vi "Sequence.BuildWaveformStep.vi"(7 "FirstIteration":bool, 9 "Current Waveform":waveform(dbl)[](array[waveform]), 10 "Steps":string[](array[string]), 11 "DataPoints":u64) -> (0 "Step Type":T1[](array[typedef]), 1 "IO Points":cluster{"Ramp Pattern":dbl[]}[](array[cluster]), 2 "iStep":bool, 3 "iStep Size":i32)   [LabVIEW 2015, in "Simple Sequence Tools - Shared.lvlib"]
uses:
  Simple Sequence Tools - Shared.lvlib
  Types/Step.Types.ctl
  <vilib>/Analysis/1siggen.llb/Ramp Pattern by Samples.vi
  <vilib>/Analysis/NI_AALBase.lvlib
  <vilib>/measure/NI_MABase.lvlib
panel:
  in  "DataPoints out":u64
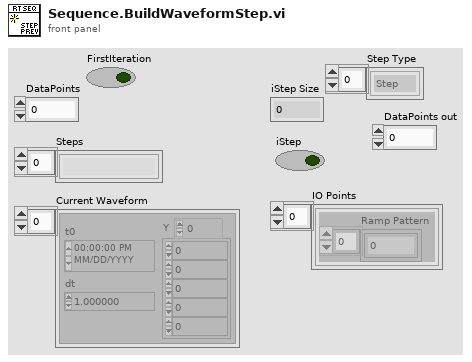
[diagram p1: front panel]
types:
  T1 = typedef "Simple Sequence Tools - Shared.lvlib/Step.Types.ctl" = enum8{"Step", "iStep", "Ramp", "Unchanged", "Unknown", "Sine", "LogSine", "LinearSine", "ForcedRamp", "SquareWave"}
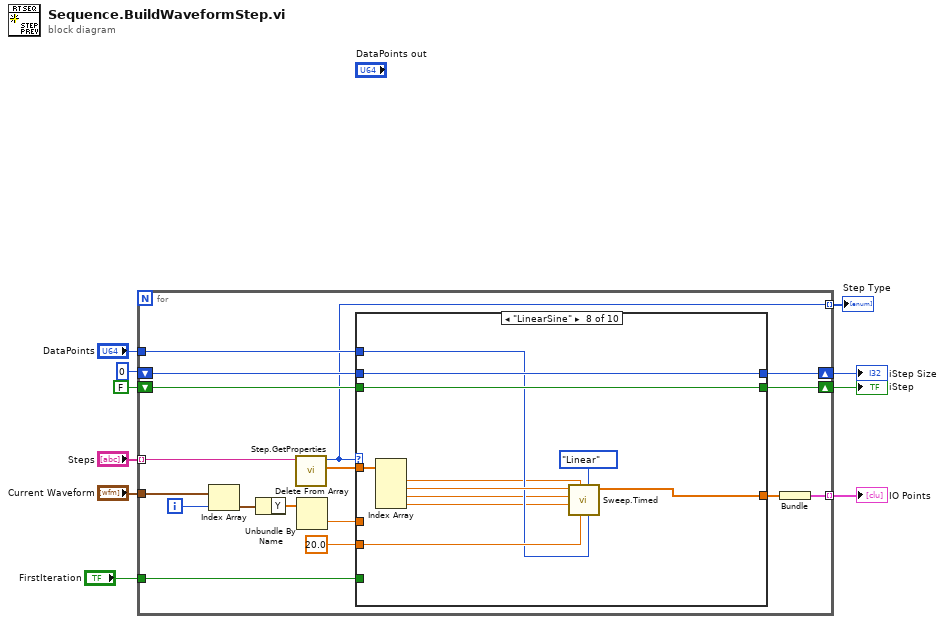
[diagram p0: block diagram]
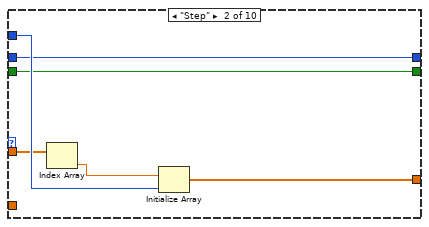
[diagram p3: hidden frame]
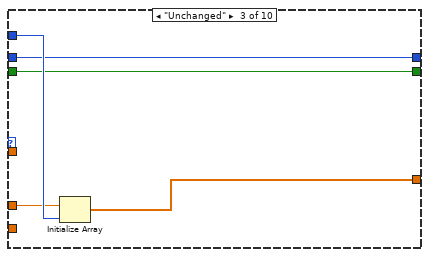
[diagram p4: hidden frame]
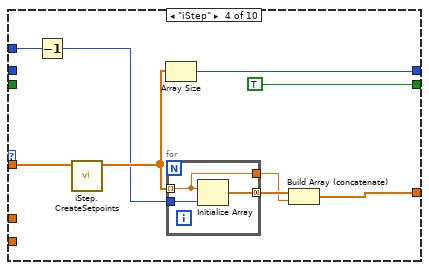
[diagram p5: hidden frame]
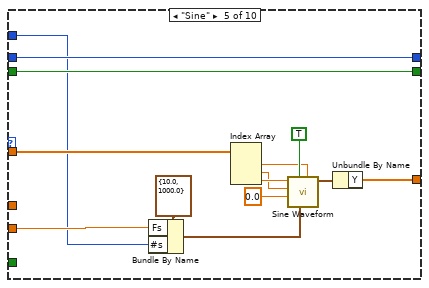
[diagram p6: hidden frame]
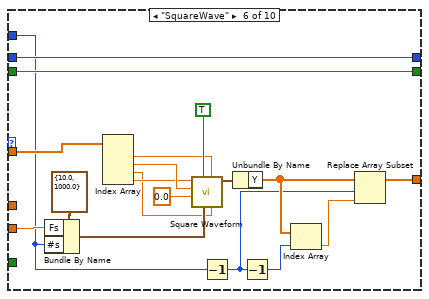
[diagram p7: hidden frame]
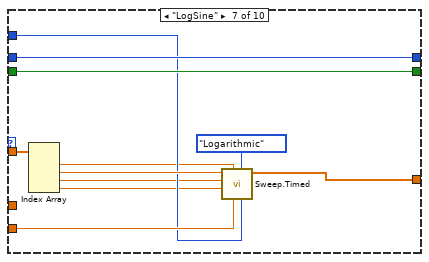
[diagram p8: hidden frame]
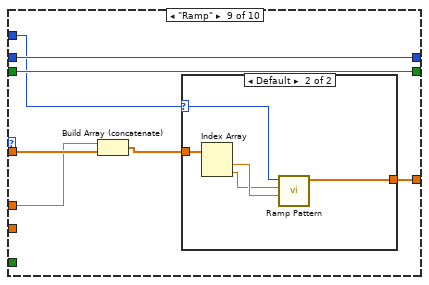
[diagram p9: hidden frame]
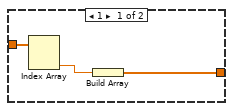
[diagram p10: hidden frame]
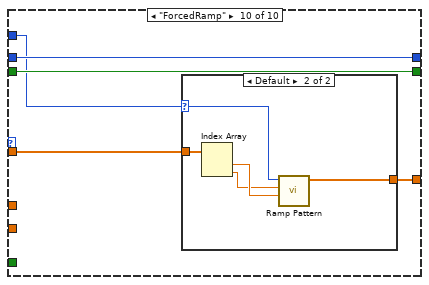
[diagram p11: hidden frame]
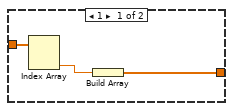
[diagram p12: hidden frame]
diagram:
  n1 = for {
    tunnel: "Steps" -> [w27] mode=indexing
    tunnel: "DataPoints" -> [w26]
    shift-right: [w23] -> w6
    shift-left: FALSE -> [w24]
    shift-right: [w21] -> w7
    shift-left: 0 -> [w20]
    tunnel: [w19] -> w8 mode=indexing
    tunnel: "Current Waveform" -> [w18]
    tunnel: [w12] -> w2 mode=indexing
    tunnel: "FirstIteration" -> [w11]
    i -> [w16]
    n2 = Index Array(array=w18, index=w16) -> (element=w15:waveform(dbl))
    n3 = Unbundle By Name(w15) -> ("Y"=w14:dbl[])
    n4 = call "Step.GetProperties.vi"("String in"=w27) -> ("Parameters"=w25:dbl[], "Step"=w12:T1)  [unwired: 8 in, 1 out]
    n5 = Delete From Array(array=w14) -> (deleted portion=w17:dbl)  [unwired: 2 in, 1 out]
    n6 = case shown="\"LinearSine\"" w12 {
      tunnel: w26 -> [_ w35 w40 w48 w53 w72 w90 w101 w111 w124]
      tunnel: w25 -> [_ w34 _ w49 w66 w85 w94 w105 w110 w123]
      tunnel: [_ w32 w39 w42 w60 w70 w91 w102 w114 w127] -> w22
      tunnel: w24 -> [w29 w31 w38 _ w55 w76 w95 w106 w113 w126]
      tunnel: [w29 w31 w38 TRUE w55 w76 w95 w106 w113 w126] -> w23
      tunnel: [w28 w30 w37 w44 w65 w84 w96 w107 w112 w125] -> w21
      tunnel: w20 -> [w28 w30 w37 _ w65 w84 w96 w107 w112 w125]
      tunnel: w17 -> [_ _ w36 _ _ _ _ _ w109 _]
      tunnel: 20.0 ("Fs") -> [_ _ _ _ w54 w75 w92 w103 _ _]
      tunnel: w11 -> [_ _ _ _ _ _ _ _ _ _]
      frame Default {
      }
      frame "Step" {
        n7 = Index Array(array=w34) -> (element=w33:dbl)  [unwired: 1 in]
        n8 = Initialize Array(w33, w35) -> (w32:dbl[])
      }
      frame "Unchanged" {
        n9 = Initialize Array(w36, w40) -> (w39:dbl[])
      }
      frame "iStep" {
        n10 = Decrement(x=w48) -> (x-1=w43:u64)
        n11 = call "iStep.CreateSetpoints.vi"("Parameters"=w49) -> ("iStep Pattern"=w45:dbl[])  [unwired: 9 in, 1 out]
        n12 = Array Size(array=w45) -> (size(s)=w44:i32)
        n13 = for {
          tunnel: w43 -> [w52]
          tunnel: w45 -> [w50] mode=indexing
          tunnel: [w51] -> w46 mode=concatenating
          tunnel: [w50] -> w41
          n14 = Initialize Array(w50, w52) -> (w51:dbl[])
        }
        n15 = Build Array (concatenate)(w46, w41) -> (w42:dbl[])
      }
      frame "Sine" {
        n16 = Bundle By Name(cluster=cluster{"Fs":dbl, "#s":dbl} {"Fs"=10.0, "#s"=1000.0} ("sampling info"), "Fs"=w54, "#s"=w53) -> (w58:cluster{"Fs":dbl, "#s":dbl})
        n17 = Index Array(array=w66) -> (element #1=w56:dbl, element #2=w57:dbl, element #3=w64:dbl)  [unwired: 3 in]
        n18 = call <vilib>:"Sine Waveform.vi"("offset"=w56, "sampling info"=w58, "reset signal"=TRUE ("reset phase"), "phase"=0.0 ("phase in"), "amplitude"=w57, "frequency"=w64) -> ("signal out"=w61:waveform(dbl))  [unwired: 4 in, 1 out]
        n19 = Unbundle By Name(w61) -> ("Y"=w60:dbl[])
      }
      frame "SquareWave" {
        n20 = Bundle By Name(cluster=cluster{"Fs":dbl, "#s":dbl} {"Fs"=10.0, "#s"=1000.0} ("sampling info"), "Fs"=w75, "#s"=w72) -> (w79:cluster{"Fs":dbl, "#s":dbl})
        n21 = Index Array(array=w85) -> (element #1=w77:dbl, element #2=w78:dbl, element #3=w73:dbl, element #4=w74:dbl)  [unwired: 4 in]
        n22 = call <vilib>:"Square Waveform.vi"("duty cycle (%)"=w73, "offset"=w77, "sampling info"=w79, "reset signal"=TRUE ("reset phase"), "phase"=0.0 ("phase in"), "amplitude"=w78, "frequency"=w74) -> ("signal out"=w81:waveform(dbl))  [unwired: 3 in, 1 out]
        n23 = Decrement(x=w72) -> (x-1=w67:u64)
        n24 = Unbundle By Name(w81) -> ("Y"=w71:dbl[])
        n25 = Decrement(x=w67) -> (x-1=w68:u64)
        n26 = Index Array(array=w71, index=w68) -> (element=w69:dbl)
        n27 = Replace Array Subset(array=w71, new element=w69, index=w67) -> (w70:dbl[])
      }
      frame "LogSine" {
        n28 = Index Array(array=w94) -> (element #1=w89:dbl, element #2=w93:dbl, element #3=w88:dbl, element #4=w87:dbl)  [unwired: 4 in]
        n29 = call "Sweep.Timed.vi"("DataPoints"=w90, "frequency spacing"=enum16{"Linear", "Logarithmic"}."Logarithmic", "Fsample (S/s)"=w92, "Offset"=w89, "EndHz"=w87, "StartHz"=w88, "Amplitude"=w93) -> ("Chirp Data"=w91:dbl[])  [unwired: 3 in, 1 out]
      }
      frame "LinearSine" {
        n30 = Index Array(array=w105) -> (element #1=w100:dbl, element #2=w104:dbl, element #3=w99:dbl, element #4=w98:dbl)  [unwired: 4 in]
        n31 = call "Sweep.Timed.vi"("DataPoints"=w101, "frequency spacing"=enum16{"Linear", "Logarithmic"}."Linear", "Fsample (S/s)"=w103, "Offset"=w100, "EndHz"=w98, "StartHz"=w99, "Amplitude"=w104) -> ("Chirp Data"=w102:dbl[])  [unwired: 3 in, 1 out]
      }
      frame "Ramp" {
        n32 = Build Array (concatenate)(w109, w110) -> (w108:dbl[])
        n33 = case shown="Default" w111 {
          selector: w111 -> [_ w121]
          tunnel: w108 -> [w117 w120]
          tunnel: [w115 w122] -> w114
          frame 1 {
            n34 = Index Array(array=w117) -> (element #2=w116:dbl)  [unwired: 2 in, 1 out]
            n35 = Build Array(w116) -> (w115:dbl[])
          }
          frame Default {
            n36 = Index Array(array=w120) -> (element #1=w119:dbl, element #2=w118:dbl)  [unwired: 2 in]
            n37 = call-poly <vilib>:"Ramp Pattern.vi"("start"=w119, "end"=w118, "samples"=w121) -> ("Ramp Pattern"=w122:dbl[])  [unwired: 7 in, 1 out]
          }
        }
      }
      frame "ForcedRamp" {
        n38 = case shown="Default" w124 {
          selector: w124 -> [_ w134]
          tunnel: w123 -> [w130 w133]
          tunnel: [w128 w135] -> w127
          frame 1 {
            n39 = Index Array(array=w130) -> (element #2=w129:dbl)  [unwired: 2 in, 1 out]
            n40 = Build Array(w129) -> (w128:dbl[])
          }
          frame Default {
            n41 = Index Array(array=w133) -> (element #1=w132:dbl, element #2=w131:dbl)  [unwired: 2 in]
            n42 = call-poly <vilib>:"Ramp Pattern.vi"("start"=w132, "end"=w131, "samples"=w134) -> ("Ramp Pattern"=w135:dbl[])  [unwired: 7 in, 1 out]
          }
        }
      }
    }
    n43 = Bundle("Ramp Pattern"=w22) -> (w19:cluster{"Ramp Pattern":dbl[]})  [unwired: 1 in]
  }
  "IO Points" <- w8
  "iStep Size" <- w7
  "iStep" <- w6
  "Step Type" <- w2
